vi "TestBuildPISLoop.vi"(8 "error in (no error)":errorcluster) -> (0 "error out":errorcluster)   [LabVIEW 2019]
uses:
  <vilib>/addons/_JKI Toolkits/Caraya/classes/Test/Test.lvclass
  <vilib>/addons/_JKI Toolkits/Caraya/classes/Assert/Assert.lvclass
  <vilib>/addons/_JKI Toolkits/Caraya/classes/Assert/Assert Equal Value_Variant.vi
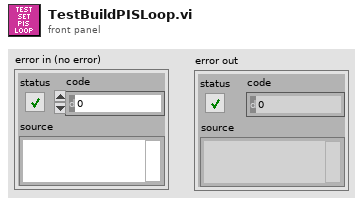
[diagram p1: front panel]
types:
  T1 = cluster{"setpoint":dbl, "pgain":dbl, "igain":dbl, "sgain":dbl}
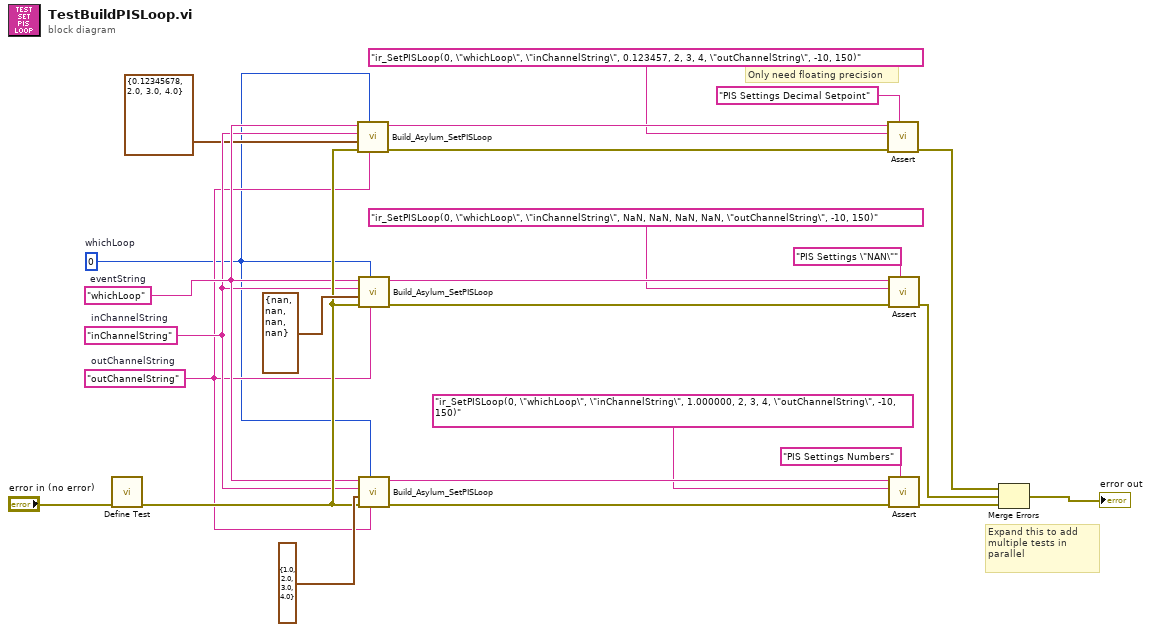
[diagram p0: block diagram]
diagram:
  w8 = "outChannelString"  # outChannelString
  w9 = "inChannelString"  # inChannelString
  w10 = "whichLoop"  # eventString
  w6 = 0  # whichLoop
  # "Only need floating precision"
  # "Expand this to add multiple tests in parallel"
  n1 = call <vilib>:"Define Test.vi"("error in (no error)"="error in (no error)") -> ("error out"=w11:errorcluster)  [unwired: 10 in]
  n2 = call "Build_Asylum_SetPISLoop.vi"("outChannelString"=w8, "whichLoop"=w6, "error in (no error)"=w11, "PIS Controls"=T1 {"setpoint"=0.12345678, "pgain"=2.0, "igain"=3.0, "sgain"=4.0}, "inChannelString"=w9, "eventString"=w10) -> ("error out"=w12:errorcluster, "Command"=w5:string)  [unwired: 4 in]
  n3 = call "Build_Asylum_SetPISLoop.vi"("outChannelString"=w8, "whichLoop"=w6, "error in (no error)"=w11, "PIS Controls"=T1 {"setpoint"=nan, "pgain"=nan, "igain"=nan, "sgain"=nan}, "inChannelString"=w9, "eventString"=w10) -> ("error out"=w18:errorcluster, "Command"=w19:string)  [unwired: 4 in]
  n4 = call "Build_Asylum_SetPISLoop.vi"("outChannelString"=w8, "whichLoop"=w6, "error in (no error)"=w11, "PIS Controls"=T1 {"setpoint"=1.0, "pgain"=2.0, "igain"=3.0, "sgain"=4.0}, "inChannelString"=w9, "eventString"=w10) -> ("error out"=w21:errorcluster, "Command"=w20:string)  [unwired: 4 in]
  n5 = call-poly <vilib>:"Assert.vi"("Label"="PIS Settings Decimal Setpoint", "error in (no error)"=w12, "Y"="ir_SetPISLoop(0, \"whichLoop\", \"inChannelString\", 0.123457, 2, 3, 4, \"outChannelString\", -10, 150)", "X"=w5) -> ("error out"=w13:errorcluster)  [unwired: 7 in]
  n6 = call-poly <vilib>:"Assert.vi"("Label"="PIS Settings \"NAN\"", "error in (no error)"=w18, "Y"="ir_SetPISLoop(0, \"whichLoop\", \"inChannelString\", NaN, NaN, NaN, NaN, \"outChannelString\", -10, 150)", "X"=w19) -> ("error out"=w16:errorcluster)  [unwired: 7 in]
  n7 = call-poly <vilib>:"Assert.vi"("Label"="PIS Settings Numbers", "error in (no error)"=w21, "Y"="ir_SetPISLoop(0, \"whichLoop\", \"inChannelString\", 1.000000, 2, 3, 4, \"outChannelString\", -10, 150)", "X"=w20) -> ("error out"=w23:errorcluster)  [unwired: 7 in]
  n8 = Merge Errors(w13, w16, w23) -> (→"error out":errorcluster)
